vi "Test Open Delphi Source.vi"   [LabVIEW 2015]
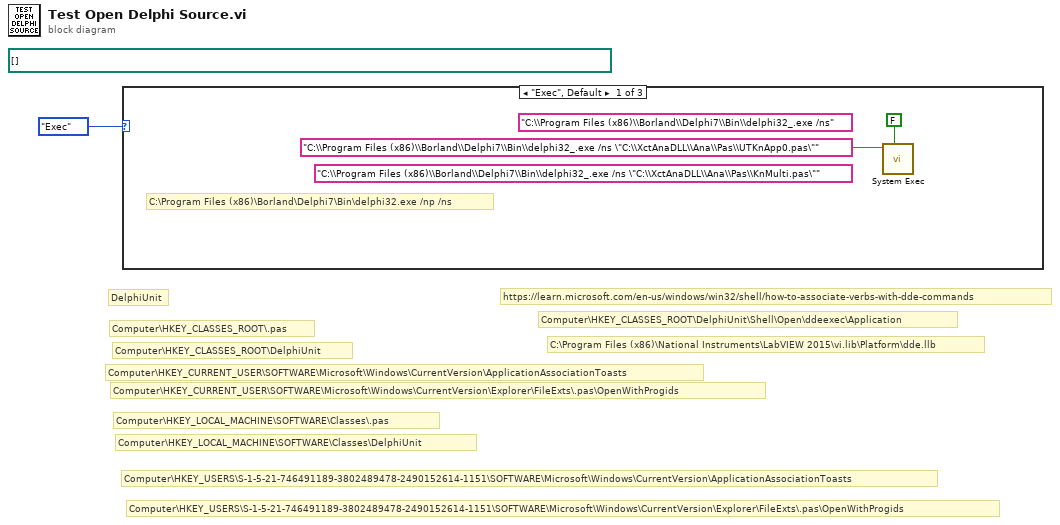
[diagram p0: block diagram]
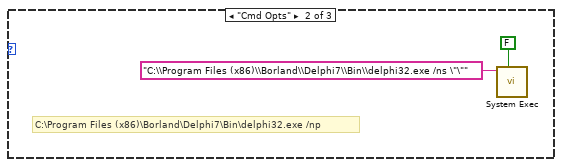
[diagram p2: hidden frame]
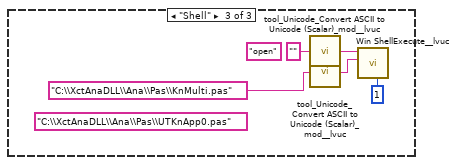
[diagram p3: hidden frame]
diagram:
  (unwired) path[] []
  # "C:\\Program Files (x86)\\National Instruments\\LabVIEW 2015\\vi.lib\\Platform\\dde.llb"
  # "Computer\\HKEY_CLASSES_ROOT\\DelphiUnit\\Shell\\Open\\ddeexec\\Application"
  # "https://learn.microsoft.com/en-us/windows/win32/shell/how-to-associate-verbs-with-dde-commands"
  # "DelphiUnit"
  # "Computer\\HKEY_CLASSES_ROOT\\DelphiUnit"
  # "Computer\\HKEY_CLASSES_ROOT\\.pas"
  # "Computer\\HKEY_USERS\\S-1-5-21-746491189-3802489478-2490152614-1151\\SOFTWARE\\Microsoft\\Windows\\CurrentVersion\\Explorer\\FileExts\\.pas\\OpenWithProgids"
  # "Computer\\HKEY_USERS\\S-1-5-21-746491189-3802489478-2490152614-1151\\SOFTWARE\\Microsoft\\Windows\\CurrentVersion\\ApplicationAssociationToasts"
  # "Computer\\HKEY_LOCAL_MACHINE\\SOFTWARE\\Classes\\DelphiUnit"
  # "Computer\\HKEY_LOCAL_MACHINE\\SOFTWARE\\Classes\\.pas"
  # "Computer\\HKEY_CURRENT_USER\\SOFTWARE\\Microsoft\\Windows\\CurrentVersion\\Explorer\\FileExts\\.pas\\OpenWithProgids"
  # "Computer\\HKEY_CURRENT_USER\\SOFTWARE\\Microsoft\\Windows\\CurrentVersion\\ApplicationAssociationToasts"
  n1 = case shown="\"Exec\", Default" enum16{"Exec", "Shell", "Cmd Opts"}."Exec" {
    frame "Exec", Default {
      (unwired) "C:\\Program Files (x86)\\Borland\\Delphi7\\Bin\\delphi32_.exe /ns" ("format string")
      (unwired) "C:\\Program Files (x86)\\Borland\\Delphi7\\Bin\\delphi32_.exe /ns \"C:\\XctAnaDLL\\Ana\\Pas\\KnMulti.pas\"" ("format string")
      # "C:\\Program Files (x86)\\Borland\\Delphi7\\Bin\\delphi32.exe /np /ns"
      n2 = call <vilib>:"System Exec.vi"("wait until completion? (T)"=FALSE, "command line"="C:\\Program Files (x86)\\Borland\\Delphi7\\Bin\\delphi32_.exe /ns \"C:\\XctAnaDLL\\Ana\\Pas\\UTKnApp0.pas\"" ("format string")) -> ()  [unwired: 6 in, 4 out]
    }
    frame "Cmd Opts" {
      # "C:\\Program Files (x86)\\Borland\\Delphi7\\Bin\\delphi32.exe /np"
      n3 = call <vilib>:"System Exec.vi"("wait until completion? (T)"=FALSE, "command line"="C:\\Program Files (x86)\\Borland\\Delphi7\\Bin\\delphi32.exe /ns \"\"" ("format string")) -> ()  [unwired: 6 in, 4 out]
    }
    frame "Shell" {
      (unwired) "C:\\XctAnaDLL\\Ana\\Pas\\UTKnApp0.pas" ("Operation (open)")
      (unwired) "open" ("Operation (open)")
      n4 = call <userlib>:"tool_Unicode_Convert ASCII to Unicode (Scalar)_mod__lvuc.vi"("ASCII"="" ("Operation (open)")) -> ("Unicode"=w9:string)  [unwired: 8 in]
      n5 = call <userlib>:"tool_Unicode_Convert ASCII to Unicode (Scalar)_mod__lvuc.vi"("ASCII"="C:\\XctAnaDLL\\Ana\\Pas\\KnMulti.pas" ("Operation (open)")) -> ("Unicode"=w10:string)  [unwired: 8 in]
      n6 = call <userlib>:"Win ShellExecute__lvuc.vi"("nShowCmd"=1, "FileW"=w10, "OperationW"=w9) -> ()  [unwired: 6 in, 3 out]
    }
  }
